vi "Initialization_of_parameters.vi"(7 "Error IN":errorcluster caption="エラー入力") -> (0 "Error OUT":errorcluster, 3 "Initial constants":T1)   [LabVIEW 2019]
panel:
  out "L":dbl
  out "l":dbl[][](array[numeric])
  out "diskofst":dbl
  out "ballangle":dbl[][](array[numeric])
  out "r":dbl
  out "q0":dbl[][](array[numeric])
  out "qmin":dbl
  out "qmax":dbl
  out "B":dbl
  out "A":dbl
  out "ArdNI_ratio":dbl
  out "distrev":dbl
  out "pulserev":dbl
  out "dt":dbl
  out "tt":dbl
  out "TT":dbl
  out "Achievable":dbl
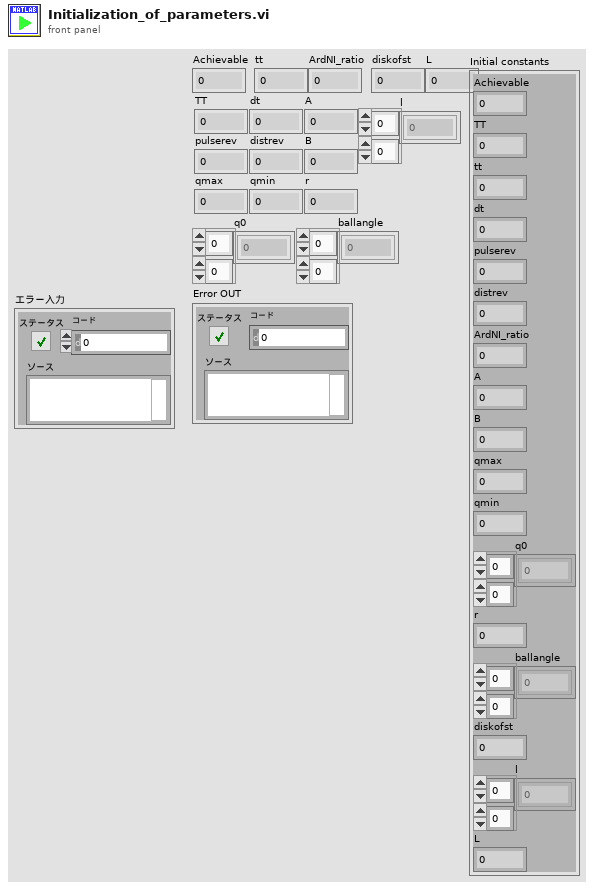
[diagram p1: front panel]
types:
  T1 = cluster{"Achievable":dbl, "TT":dbl, "tt":dbl, "dt":dbl, "pulserev":dbl, "distrev":dbl, "ArdNI_ratio":dbl, "A":dbl, "B":dbl, "qmax":dbl, "qmin":dbl, "q0":dbl[][], "r":dbl, "ballangle":dbl[][], "diskofst":dbl, "l":dbl[][], "L":dbl}
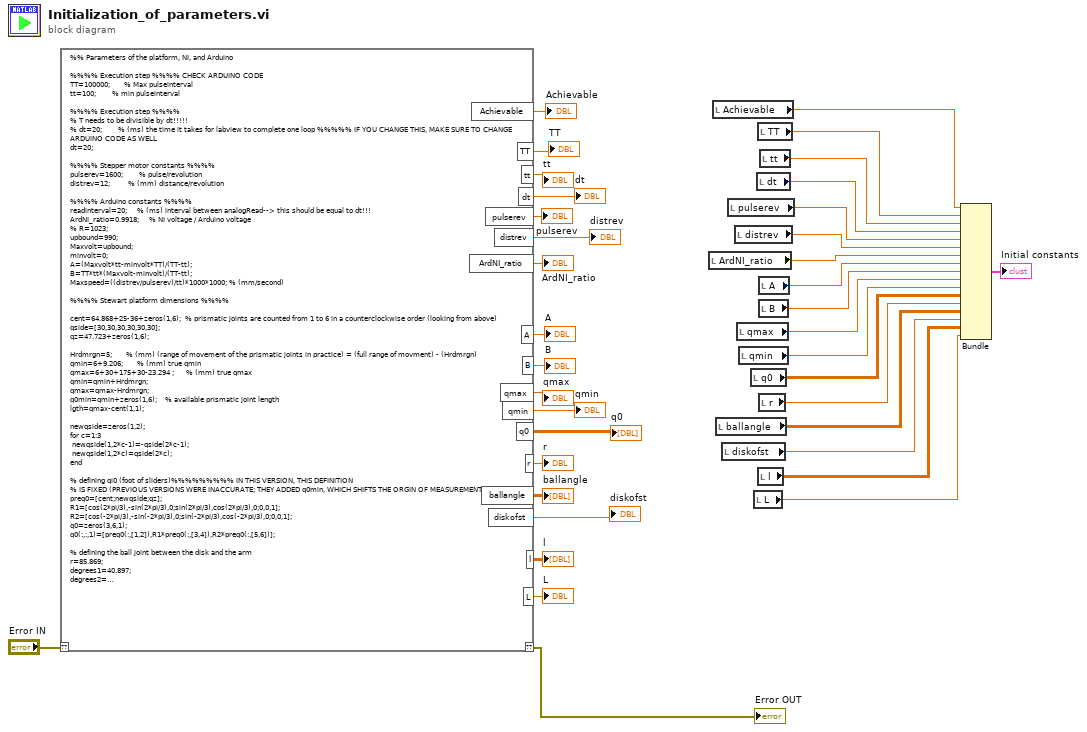
[diagram p0: block diagram]
diagram:
  n1 = script code="%% Parameters of the platform, NI, and Arduino\n\n%%%% Execution step %%%% CHECK ARDUINO CODE\nTT=100000;\t\t\t\t\t\t\t% Max pulseinterval\ntt=100;\t\t\t\t\t\t\t\t% min pulseinterval\n\n%%%% Execution step %%%%\n% T needs to be divisible by dt!!!!!\n% dt=20;\t\t\t\t\t\t\t\t% (ms) the time it takes for labview to complete one loop %%%%% IF YOU CHANGE THIS, MAKE SURE TO CHANGE ARDUINO CODE AS WELL\ndt=20;\n\n%%%% Stepper motor constants %%%%\npulserev=1600;\t\t\t\t\t\t\t\t% pulse/revolution\ndistrev=12;\t\t\t\t\t\t\t\t\t% (mm) distance/revolution\n\n%%%% Arduino constants %%%%\nreadinterval=20;\t\t\t\t\t% (ms) interval between analogRead--> this should be equal to dt!!!\nArdNI_ratio=0.9918;\t\t\t\t\t% NI voltage / Arduino voltage\n% R=1023;\nupbound=990;\nMaxvolt=upbound;\nminvolt=0;\nA=(Maxvolt*tt-minvolt*TT)/(TT-tt);\nB=TT*tt*(Maxvolt-minvolt)/(TT-tt);\nMaxspeed=((distrev/pulserev)/tt)*1000*1000;\t% (mm/second)\n\n%%%% Stewart platform dimensions %%%%\n\ncent=64.868+25-36+zeros(1,6);\t\t% prismatic joints are counted from 1 to 6 in a counterclockwise order (looking from above)\nqside=[30,30,30,30,30,30];\nqz=47.723+zeros(1,6);\n\nHrdmrgn=5;\t\t\t\t\t\t\t% (mm) (range of movement of the prismatic joints in practice) = (full range of movment) - (Hrdmrgn) \nqmin=6+9.206;\t\t\t\t\t\t\t% (mm) true qmin\nqmax=6+30+175+30-23.294 ;\t\t\t\t\t\t% (mm) true qmax\nqmin=qmin+Hrdmrgn;\nqmax=qmax-Hrdmrgn;\nq0min=qmin+zeros(1,6);\t\t\t\t% available prismatic joint length\nlgth=qmax-cent(1,1);\n\nnewqside=zeros(1,2);\nfor c=1:3\n\tnewqside(1,2*c-1)=-qside(2*c-1);\n\tnewqside(1,2*c)=qside(2*c);\nend\n\n% defining qi0 (foot of sliders)%%%%%%%%% IN THIS VERSION, THIS DEFINITION\n% IS FIXED (PREVIOUS VERSIONS WERE INACCURATE; THEY ADDED q0min, WHICH SHIFTS THE ORGIN OF MEASUREMENT)\npreq0=[cent;newqside;qz];\nR1=[cos(2*pi/3),-sin(2*pi/3),0;sin(2*pi/3),cos(2*pi/3),0;0,0,1];\nR2=[cos(-2*pi/3),-sin(-2*pi/3),0;sin(-2*pi/3),cos(-2*pi/3),0;0,0,1];\nq0=zeros(3,6,1);\nq0(:,:,1)=[preq0(:,[1,2]),R1*preq0(:,[3,4]),R2*preq0(:,[5,6])];\n\n% defining the ball joint between the disk and the arm\nr=85.869; \ndegrees1=40.897;\ndegrees2=79.103;\nradians1=deg2rad(degrees1);\nradians2=deg2rad(degrees2);\nballangle=zeros(1,6,1);\nballangle0=[-radians1/2,radians1/2,radians1/2+radians2,radians1/2+radians2+radians1,2*pi-(radians1/2+radians2+radians1),2*pi-(radians1/2+radians2)];\nballangle(1,:,1)=ballangle0;\n\n% distance between the disk surface and the center of balls\ndiskofst=10+15.458;\n\n% prismatic joint vector\nl=[];\t\t\t% (3,6)\nl(:,[1,3,5])=[1,0,0;cos(2*pi/3),sin(2*pi/3),0;cos(4*pi/3),sin(4*pi/3),0]';\nl(:,[2,4,6])=[1,0,0;cos(2*pi/3),sin(2*pi/3),0;cos(4*pi/3),sin(4*pi/3),0]';\n\n\n% arm length\nL=196; % the radius of the magnetic ball is 0.5 cm\n\nAchievable=1;"("??"="Error IN") -> ("??"=→"Error OUT":errorcluster, "TT"=→"TT":dbl, "tt"=→"tt":dbl, "dt"=→"dt":dbl, "pulserev"=→"pulserev":dbl, "distrev"=→"distrev":dbl, "ArdNI_ratio"=→"ArdNI_ratio":dbl, "A"=→"A":dbl, "B"=→"B":dbl, "qmax"=→"qmax":dbl, "qmin"=→"qmin":dbl, "q0"=→"q0":dbl[][], "r"=→"r":dbl, "ballangle"=→"ballangle":dbl[][], "diskofst"=→"diskofst":dbl, "l"=→"l":dbl[][], "L"=→"L":dbl, "Achievable"=→"Achievable":dbl)
  n2 = local read "ArdNI_ratio"() -> (w14:dbl)
  n3 = local read "Achievable"() -> (w20:dbl)
  n4 = local read "ballangle"() -> (w7:dbl[][])
  n5 = local read "diskofst"() -> (w6:dbl)
  n6 = local read "pulserev"() -> (w16:dbl)
  n7 = local read "distrev"() -> (w15:dbl)
  n8 = local read "qmax"() -> (w11:dbl)
  n9 = local read "qmin"() -> (w10:dbl)
  n10 = local read "q0"() -> (w9:dbl[][])
  n11 = local read "L"() -> (w4:dbl)
  n12 = local read "dt"() -> (w17:dbl)
  n13 = local read "TT"() -> (w19:dbl)
  n14 = local read "l"() -> (w5:dbl[][])
  n15 = local read "A"() -> (w13:dbl)
  n16 = local read "B"() -> (w12:dbl)
  n17 = local read "r"() -> (w8:dbl)
  n18 = local read "tt"() -> (w18:dbl)
  n19 = Bundle("Achievable"=w20, "TT"=w19, "tt"=w18, "dt"=w17, "pulserev"=w16, "distrev"=w15, "ArdNI_ratio"=w14, "A"=w13, "B"=w12, "qmax"=w11, "qmin"=w10, "q0"=w9, "r"=w8, "ballangle"=w7, "diskofst"=w6, "l"=w5, "L"=w4) -> (→"Initial constants":T1)  [unwired: 1 in]
